vi "Get_DIO_Devices.vi"(8 "error in (no error)":errorcluster, 10 "Direction":T1, 11 "Device":tag) -> (0 "error out":errorcluster, 2 "Lines":tag[](array[tag]), 3 "Devices":tag[](array[tag]))   [LabVIEW 2021, in "DAQmx.lvlib"]
uses:
  DAQmx.lvlib
  Dependencies/DIO-Channel.lvlibp/Channels/DIO-Channel/DIO-Configuration_class/tdef/Direction.ctl
  <resource>/objmgr/daqmx.rc
  Dependencies/DIO-Channel.lvlibp/Channels/DIO-Channel/DIO-Configuration_class/DIO-Configuration.lvclass
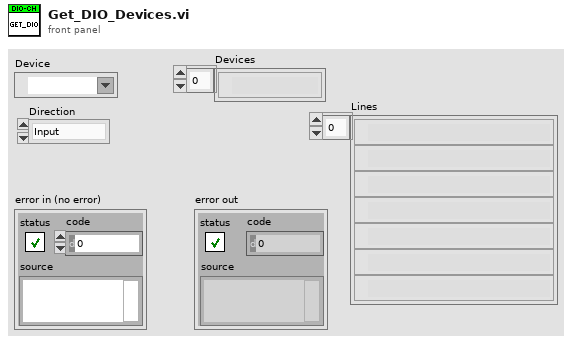
[diagram p1: front panel]
types:
  T1 = typedef "DIO-Channel.lvlibp/DIO-Configuration.lvclass/Direction.ctl" = enum16{"Input", "Output"}
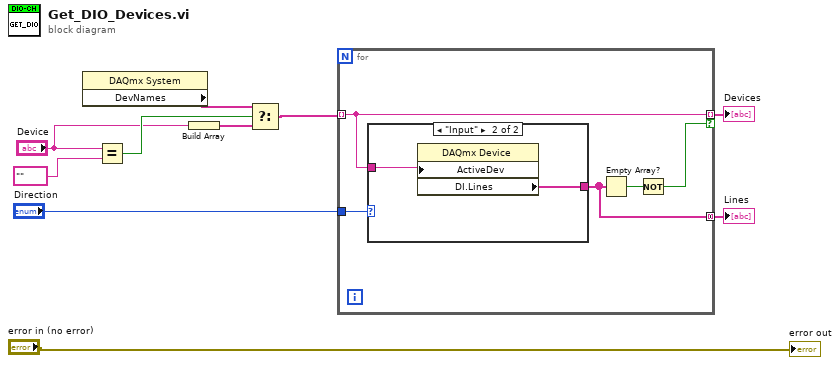
[diagram p0: block diagram]
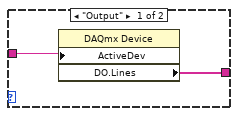
[diagram p2: hidden frame]
diagram:
  n1 = property class="DAQmx System"() -> ("DevNames"=w10:tag[])  [unwired: 2 in, 2 out]
  n2 = Equal?(x="Device", y=tag "" ("Device")) -> (x = y?=w4:bool)
  n3 = Build Array("Device") -> (w3:tag[])
  n4 = Select(t=w10, s=w4, f=w3) -> (s? t:f=w5:tag[])
  n5 = for {
    tunnel: w5 -> [w14] mode=indexing
    tunnel: "Direction" -> [w15]
    tunnel: [w14] -> w8 mode=indexing if=w11
    tunnel: [w12] -> w7 mode=concatenating
    n6 = case shown="\"Input\"" w15 {
      tunnel: w14 -> [w17 w19]
      tunnel: [w16 w18] -> w12
      frame "Output" {
        n7 = property class="DAQmx Device"("ActiveDev"=w17) -> ("DO.Lines"=w16:tag[])  [unwired: 2 in, 2 out]
      }
      frame "Input" {
        n8 = property class="DAQmx Device"("ActiveDev"=w19) -> ("DI.Lines"=w18:tag[])  [unwired: 2 in, 2 out]
      }
    }
    n9 = Empty Array?(array=w12) -> (empty?=w13:bool)
    n10 = Not(x=w13) -> (.not. x?=w11:bool)
  }
  "Devices" <- w8
  "Lines" <- w7
  "error out" <- "error in (no error)"
